vi "CSE - Execute Parsed Script.vi"(6 "exec parameters":T2={"pause counter"=1000, "pause, ms"=0, "autoVar"=TRUE, "enCpx"=TRUE}, 7 "VC Handle":T4=-1, 8 "error in":errorcluster, 9 "Close FuncVI Refs (T)":bool=TRUE, 10 "Callback VI RefNum":T1, 11 "CSE RefNum":T3) -> (0 "error out":errorcluster, 1 "return value":dbl, 2 "dup Callback VI RefNum":T1, 3 "dup CSE RefNum":T3, 5 "dup VC Handle":T4=-1)   [LabVIEW 2021]
doc: "The VI executes a parsed CSE script. Refer to the VI help for more details.\n\n<b>CSE RefNum</b> must contain a reference to a CSE instance context containing a parsed script.\n\n<b>VC Handle</b> specifies the handle of a variable context. CalcExpress accesses variables using this handle.\n\n<b>return value</b> indicates the value of the <b>return</b> statement in a script.\n\n::: CalcExpress Toolkit :::\nCopyright (c) 2000-2026 Konstantin Shifershteyn. All rights reserved."
uses:
  cetypes.llb/VarMan Variable Context Handle.ctl
  CSE Instance RefNum.ctl
  cetypes.llb/CSE Execution Options.ctl
  CSE Callback VI RefNum.ctl
  CSE Type - Callback Call Reason.ctl
  CSE Type - Run Mode.ctl
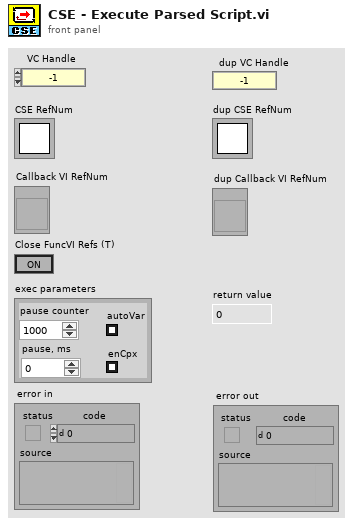
[diagram p1: front panel]
types:
  T1 = typedef "CSE Callback VI RefNum.ctl" = refnum<vi>
  T2 = typedef "CSE Execution Options.ctl" = cluster{"pause counter":i32, "pause, ms":i32, "autoVar":bool, "enCpx":bool}
  T3 = typedef "CSE Instance RefNum.ctl" = refnum<k1>
  T4 = typedef "VarMan Variable Context Handle.ctl" = i32
  T5 = typedef "CSE Type - Callback Call Reason.ctl" = u32
  T6 = enum32{"nothing", "reset", "assign name", "get name", "get handle"}
  T7 = typedef "CSE Type - Run Mode.ctl" = u32
  T8 = enum16{"get RefNum", "close Clones", "close RefNum", "close all RefNums", "update RefNums"}
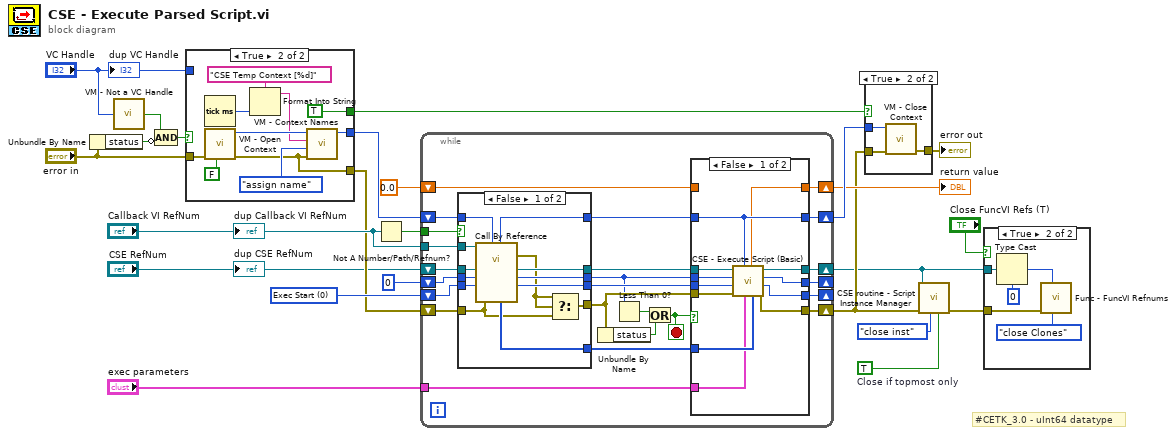
[diagram p0: block diagram]
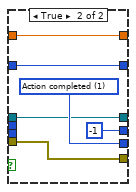
[diagram p3: hidden frame]
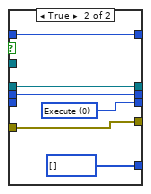
[diagram p4: hidden frame]
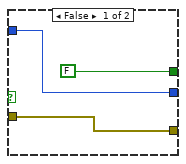
[diagram p6: hidden frame]
diagram:
  w2 = TRUE  # Close if topmost only
  w11 = T5 0 items=["Exec Start", "Action completed", "pause to breath", "reserved 1", "reserved 2", "custom"] ("Call Reason")
  # "#CETK_3.0 - uInt64 datatype"
  n1 = Unbundle By Name("error in") -> ("status"=w21:bool)
  n2 = call "VM - Not a VC Handle.vi"("VC Handle"="VC Handle") -> ("Not a VC Handle"=w19:bool)  [unwired: 1 in]
  n3 = Compound Arithmetic op=AND(w19, invert w21) -> (w20:bool)
  n4 = case shown="True" w20 {
    tunnel: [w27 w32] -> w9
    tunnel: "error in" -> [w27 w36]
    tunnel: [w25 w33] -> w16
    tunnel: [FALSE TRUE] -> w24
    tunnel: "VC Handle" -> [w25 _]
    frame False {
    }
    frame True {
      n5 = Tick Count (ms)() -> (millisecond timer value=w30:u32)
      n6 = call "VM - Open Context.vi"("close loose contexts (F)"=FALSE ("close loose contexts (T)"), "error in"=w36) -> ("error out"=w32:errorcluster, "VC Handle out"=w34:T4)  [unwired: 7 in, 1 out]
      n7 = Format Into String(format string="CSE Temp Context [%d]", w30) -> (resulting string=w29:string)  [unwired: 2 in, 1 out]
      n8 = call "VM - Context Names.vi"("error in"=w32, "action"=T6."assign name", "VC Name"=w29, "VC Handle"=w34) -> ("VC Handle out"=w33:T4)  [unwired: 2 in, 3 out]
    }
  }
  n9 = Not A Number/Path/Refnum?(number/path/refnum="Callback VI RefNum") -> (NaN/Path/Refnum?=w12:bool)
  n10 = while {
    shift-right: [w61] -> w6
    shift-left: w9 -> [w55]
    shift-right: [w47] -> w15
    shift-left: w16 -> [w48]
    shift-right: [w60] -> _
    shift-left: 0 ("Stm Index out") -> [w58]
    tunnel: w12 -> [w54]
    shift-right: [w41] -> _
    shift-left: w11 -> [w42]
    shift-right: [w44] -> w14
    shift-left: 0.0 ("return value") -> [w43]
    tunnel: "Callback VI RefNum" -> [w40]
    shift-right: [w39] -> w4
    shift-left: "CSE RefNum" -> [w59]
    tunnel: "exec parameters" -> [w38]
    stop <- w49 stop-if-true
    n11 = case shown="False" w54 {
      tunnel: w59 -> [w91 w98]
      tunnel: w58 -> [w90 w97]
      tunnel: [w86 w98] -> w57
      tunnel: [w85 w97] -> w52
      tunnel: [w84 w93] -> w56
      tunnel: w55 -> [w81 w96]
      tunnel: [w80 w96] -> w53
      tunnel: w48 -> [w88 w95]
      tunnel: [w87 w95] -> w46
      tunnel: [w83 i32[] [] ("BreakPoints")] -> w45
      tunnel: w42 -> [w89 _]
      tunnel: w40 -> [w92 _]
      frame False {
        n12 = call-by-ref "?"(reference=w92, "VC Handle"=w88, "error in"=w81, "Call Reason"=w89, "Stm Index"=w90, "CSE RefNum"=w91) -> (error out=w82:errorcluster, "Run Mode"=w84:T7, "Stm Index out"=w85:i32, "dup CSE RefNum"=w86:T3, "Breakpoints"=w83:i32[], "VC Handle out"=w87:T4)  [unwired: 2 in, 2 out]
        n13 = Select(t=w82, s=w82, f=w81) -> (s? t:f=w80:errorcluster)
      }
      frame True {
        w93 = T7 0 items=["Execute", "Abort", "Run", "Step", "Step Over", "Step Out", "Run (LM)", "Step (LM)", "Step Over (LM)", "Step Out (LM)", "unsupported"] ("Run mode")
      }
    }
    n14 = Unbundle By Name(w53) -> ("status"=w50:bool)
    n15 = Less Than 0?(x=w52) -> (x < 0?=w51:bool)
    n16 = Or(x=w51, y=w50) -> (x .or. y?=w49:bool)
    n17 = case shown="False" w49 {
      tunnel: [w73 w78] -> w61
      tunnel: [w72 -1 ("Stm Index out")] -> w60
      tunnel: w57 -> [w71 w74]
      tunnel: w52 -> [w70 _]
      tunnel: w56 -> [w69 _]
      tunnel: w53 -> [w68 w78]
      tunnel: [w67 w77] -> w47
      tunnel: w46 -> [w67 w77]
      tunnel: w45 -> [w66 _]
      tunnel: [w65 w76] -> w44
      tunnel: w43 -> [_ w76]
      tunnel: [w64 w75] -> w41
      tunnel: [w63 w74] -> w39
      tunnel: w38 -> [w62 _]
      frame False {
        n18 = call "CSE - Execute Script (Basic).vi"("Breakpoints"=w66, "exec parameters"=w62, "VC Handle"=w67, "error in"=w68, "Run mode"=w69, "Stm Index"=w70, "CSE RefNum"=w71) -> ("error out"=w73:errorcluster, "Stop Reason"=w64:T5, "Stm Index out"=w72:i32, "dup CSE RefNum"=w63:T3, "return value"=w65:dbl)
      }
      frame True {
        w75 = T5 1 items=["Exec Start", "Action completed", "pause to breath", "reserved 1", "reserved 2", "custom"] ("Call Reason")
      }
    }
  }
  "return value" <- w14
  n19 = case shown="True" w24 {
    tunnel: w15 -> [_ w102]
    tunnel: w6 -> [w99 w101]
    tunnel: [w99 w100] -> w23
    frame False {
    }
    frame True {
      n20 = call "VM - Close Context.vi"("error in"=w101, "VC Handle"=w102) -> ("error out"=w100:errorcluster)  [unwired: 8 in, 1 out]
    }
  }
  "error out" <- w23
  n21 = call "CSE routine - Script Instance Manager.vi"("Close if topmost only (f)"=w2, "cmd (open)"=enum16{"open", "close inst", "close all"}."close inst" ("cmd (get)"), "error in"=w6, "Caller CSE RefNum"=w4) -> ("error out"=w5:errorcluster)  [unwired: 5 in, 2 out]
  n22 = case shown="True" "Close FuncVI Refs (T)" {
    tunnel: w4 -> [_ w106]
    tunnel: w5 -> [_ w105]
    frame False {
    }
    frame True {
      n23 = Type Cast(type=u64 0, x=w106) -> (*(type *) &x=w104:u64)
      n24 = call "Func - FuncVI Refnums.vi"("cmd (get)"=T8."close Clones", "Instance ID"=w104, "error in"=w105) -> ()  [unwired: 4 in, 5 out]
    }
  }
  "dup VC Handle" <- "VC Handle"
  "dup CSE RefNum" <- "CSE RefNum"
  "dup Callback VI RefNum" <- "Callback VI RefNum"
